vi "Add Control Details To Schema.vi"(8 "error in":errorcluster, 9 "required?":bool, 10 "control":refnum<vi>, 11 "schema":string) -> (0 "error out":errorcluster, 3 "schema out":string)   [LabVIEW 2020, in "MCP Server.lvlib"]
doc: "Adds what the front panel control of a tool input says beyond its type to the JSON Schema of that input, for tools/list. Wire the schema LV Type To JSON Schema.vi made for the control's type into schema, and the control itself into control. The control and its elements are walked together with the schema, to any depth (clusters by element label under properties, array elements under items): every element with a description gets it as description (except LabVIEW's default error cluster descriptions, which Remove Default Error Description.vi leaves out), integers get minimum and maximum from their representation (I8 -128 to 127 up to U64 0 to 18446744073709551615, written as exact integers), a numeric whose data entry limits are not set to Ignore gets those limits instead where they are tighter, and a numeric with a unit gets \"Unit: <unit>.\" appended to its description. The control itself only gets a description when it has a unit (tool list.vi takes its description from the control otherwise), and, when the input is not required, its default value as default, serialized with JSONtext like tools/call values (left out above 1024 characters). Details that cannot be read from a control are left out. With an error in, or without a valid control, schema is passed through unchanged."
uses:
  MCP Server.lvlib
  <vilib>/JDP Science/JSONtext/Next JSON Value.vi
  <vilib>/JDP Science/JSONtext/String Subset.vi
  <vilib>/JDP Science/JSONtext/Parsing/Advance past next JSON Value (inlined COPY).vi
  <vilib>/JDP Science/JSONtext/Parsing/Advance past whitespace.vi
  <vilib>/JDP Science/JSONtext/Parsing/Advance past String.vi
  <vilib>/JDP Science/JSONtext/Parsing/Advance past Number.vi
  <vilib>/JDP Science/JSONtext/Parsing/Advance past Line Ending.vi
  <vilib>/JDP Science/JSONtext/Parsing/Parse Full Path or Item Name.vi
  <vilib>/JDP Science/JSONtext/Parsing/Advance past Array.vi
  <vilib>/JDP Science/JSONtext/Parsing/Advance past Object.vi
  <vilib>/JDP Science/JSONtext/support/Error Cluster From Code.vi
  <vilib>/JDP Science/JSONtext/Offset/Find Item Locations by Path.vi
  <vilib>/JDP Science/JSONtext/Get all Object Items.vi
  <vilib>/JDP Science/JSONtext/Set Multiple Object Items.vi
  <vilib>/JDP Science/JSONtext/JSONtext.lvlib
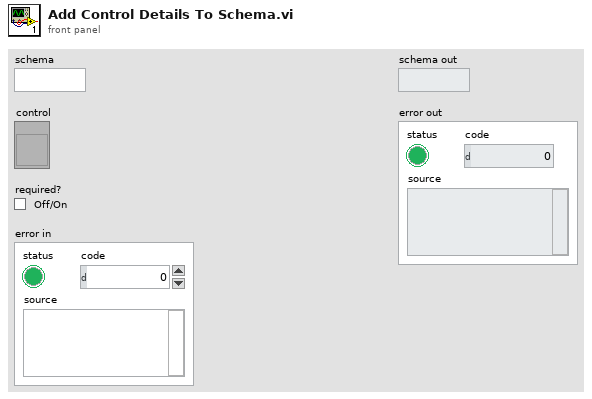
[diagram p1: front panel]
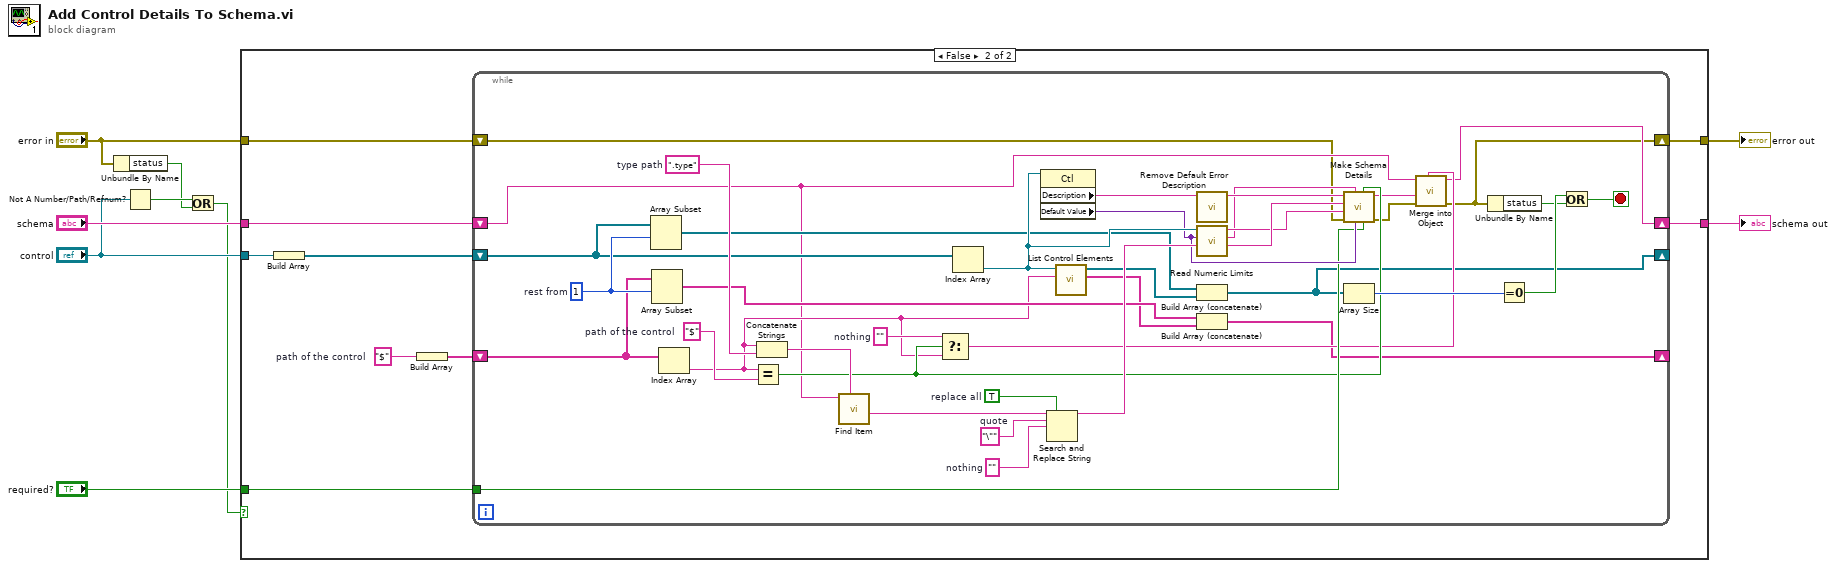
[diagram p0: block diagram]
diagram:
  n1 = Unbundle By Name("error in") -> ("status"=w8:bool)
  n2 = Not A Number/Path/Refnum?(number/path/refnum="control") -> (NaN/Path/Refnum?=w9:bool)
  n3 = Or(x=w9, y=w8) -> (x .or. y?=w3:bool)
  n4 = case shown="False" w3 {
    tunnel: "schema" -> [w11 w15]
    tunnel: "control" -> [_ w20]
    tunnel: "required?" -> [_ w18]
    tunnel: "error in" -> [w10 w14]
    tunnel: [w11 w13] -> w2
    tunnel: [w10 w12] -> w1
    frame True {
    }
    frame False {
      w19 = "$"  # path of the control
      n5 = Build Array(w20) -> (w17:refnum<vi>[])
      n6 = Build Array(w19) -> (w16:string[])
      n7 = while {
        tunnel: w18 -> [w43]
        shift-right: [w28] -> _
        shift-left: w17 -> [w27]
        shift-right: [w26] -> _
        shift-left: w16 -> [w25]
        shift-right: [w24] -> w13
        shift-left: w15 -> [w23]
        shift-right: [w22] -> w12
        shift-left: w14 -> [w21]
        stop <- w29 stop-if-true
        w37 = ""  # nothing
        w51 = TRUE  # replace all
        w52 = ""  # nothing
        w53 = "\""  # quote
        w57 = ".type"  # type path
        w58 = "$"  # path of the control
        w59 = 1  # rest from
        n8 = Array Subset(array=w27, index=w59) -> (w42:refnum<vi>[])  [unwired: 1 in]
        n9 = Array Subset(array=w25, index=w59) -> (w40:string[])  [unwired: 1 in]
        n10 = Index Array(array=w25) -> (element=w35:string)  [unwired: 1 in]
        n11 = Equal?(x=w35, y=w58) -> (x = y?=w36:bool)
        n12 = Concatenate Strings(w35, w57) -> (w55:string)
        n13 = call <vilib>:"Find Item.vi"("$Path or Item Name"=w55, "JSON"=w23) -> ("<JSON>"=w54:string)  [unwired: 6 in, 3 out]
        n14 = Select(t=w37, s=w36, f=w35) -> (s? t:f=w32:string)
        n15 = Index Array(array=w27) -> (element=w50:refnum<vi>)  [unwired: 1 in]
        n16 = property class="Ctl"(reference=w50) -> ("Description"=w56:string, "Default Value"=w44:variant)  [unwired: 1 in, 2 out]
        n17 = Search and Replace String(replace all?=w51, input string=w54, search string=w53, replace string=w52) -> (result string=w49:string)  [unwired: 4 in, 3 out]
        n18 = call "List Control Elements.vi"("path"=w35, "control"=w50) -> ("element paths"=w39:string[], "element controls"=w41:refnum<vi>[])  [unwired: 8 in]
        n19 = call "Remove Default Error Description.vi"("description"=w56) -> ("description out"=w48:string)  [unwired: 10 in]
        n20 = call "Read Numeric Limits.vi"("schema type"=w49, "default value"=w44, "control"=w50) -> ("unit note"=w47:string, "maximum"=w45:string, "minimum"=w46:string)  [unwired: 6 in]
        n21 = Build Array (concatenate)(w42, w41) -> (w28:refnum<vi>[])
        n22 = Build Array (concatenate)(w40, w39) -> (w26:string[])
        n23 = call "Make Schema Details.vi"("required?"=w43, "control itself?"=w36, "default value"=w44, "maximum"=w45, "error in"=w21, "minimum"=w46, "unit note"=w47, "description"=w48) -> ("error out"=w33:errorcluster, "details"=w34:string)  [unwired: 2 in]
        n24 = Array Size(array=w28) -> (size(s)=w38:i32)
        n25 = call <vilib>:"Merge into Object.vi"("$Path or Item Name"=w32, "error in (no error)"=w33, "JSON Object to Merge"=w34, "JSON"=w23) -> ("error out"=w22:errorcluster, "<JSON>"=w24:string)  [unwired: 5 in]
        n26 = Unbundle By Name(w22) -> ("status"=w30:bool)
        n27 = Equal To 0?(x=w38) -> (x = 0?=w31:bool)
        n28 = Or(x=w31, y=w30) -> (x .or. y?=w29:bool)
      }
    }
  }
  "schema out" <- w2
  "error out" <- w1
